vi "Complete Request.vi"(7 "Processing In":refnum<class "Processing.lvclass">, 11 "Session Cleanup Handler in":refnum<class "Session Cleanup Handler.lvclass">) -> (0 "error out":errorcluster, 5 "Processing":refnum<class "Processing.lvclass">)   [LabVIEW 2020, in "HTTP Server.lvlib" / "Session Cleanup Handler.lvclass"]
uses:
  Session Cleanup Handler.lvclass
  Processing/Processing.lvclass
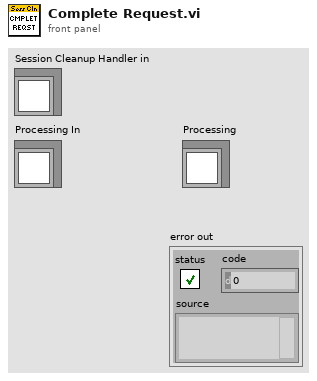
[diagram p1: front panel]
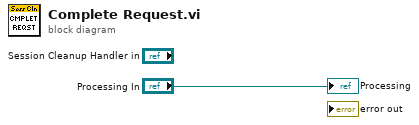
[diagram p0: block diagram]
diagram:
  "Processing" <- "Processing In"
